vi "MCLB_FocusIndexArray_Tests.vi"(11 "error in":errorcluster) -> (15 "error out":errorcluster)   [LabVIEW 2016, in "DronaTest.lvlib"]
uses:
  DronaTest.lvlib
  APIs/Stimulus/ControlValue/SetValueAuto.vi
  APIs/Stimulus/ControlValue/Controls/MC Listbox/SetValueByArrayIndex.vi
  APIs/Assert/AssertControlValue/Controls/MC Listbox/AssertValueByArrayIndex.vi
  <vilib>/addons/_JKI Toolkits/Caraya/classes/Assert/Assert Error.vi
  <vilib>/addons/_JKI Toolkits/Caraya/classes/Assert/Assert Equal Value_Variant.vi
  <vilib>/addons/_JKI Toolkits/Caraya/classes/Test/Test.lvclass
  Drona.lvlib
  <vilib>/SLL Toolkit/SLL Debug/SLL Debug.lvlib
  <vilib>/addons/_JKI Toolkits/Caraya/classes/Assert/Assert.lvclass
  APIs/Stimulus/ControlValue/Controls/MC Listbox/StimulusMCListbox.lvlib
  APIs/Assert/AssertControlValue/Controls/MC Listbox/AssertMCListbox.lvlib
  APIs/Stimulus/ControlValue/ControlValue.lvlib
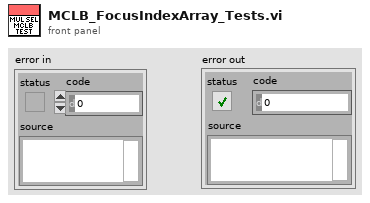
[diagram p1: front panel]
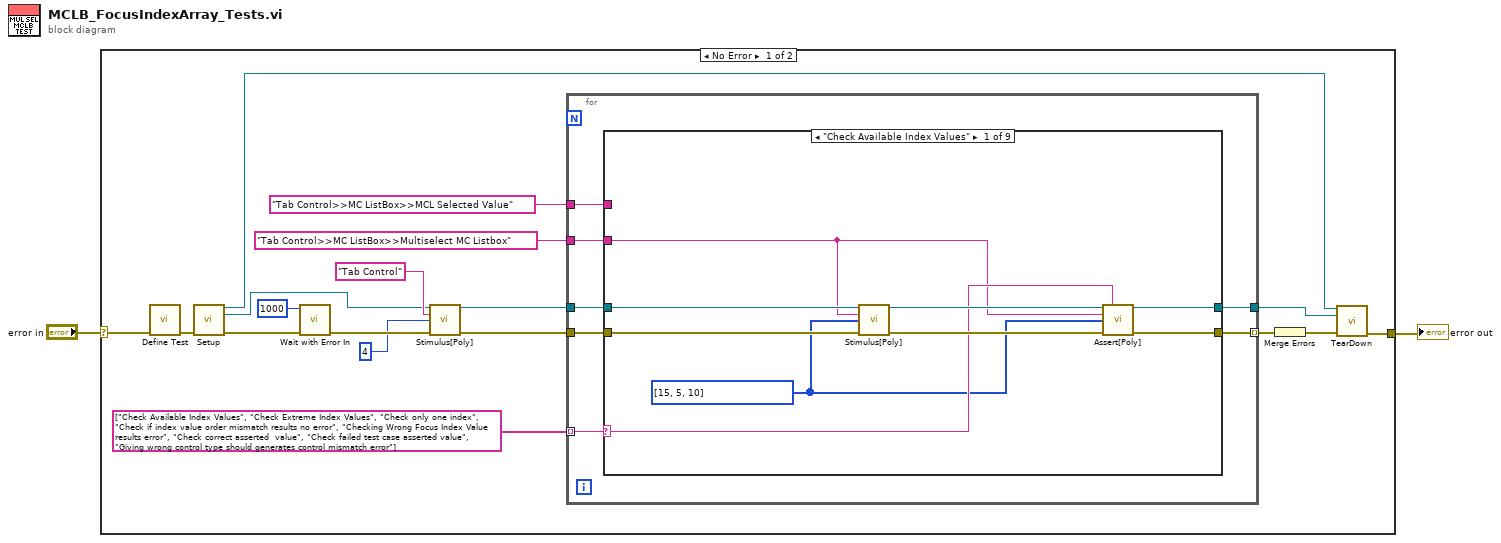
[diagram p0: block diagram]
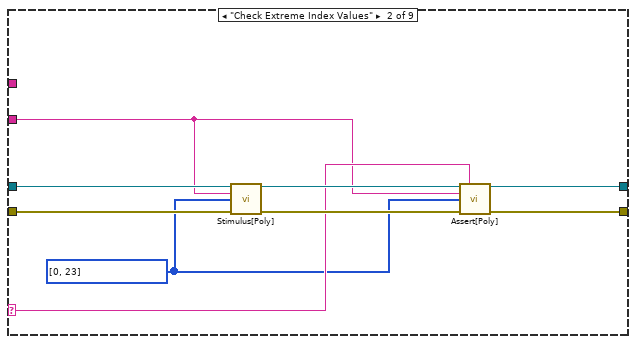
[diagram p2: hidden frame]
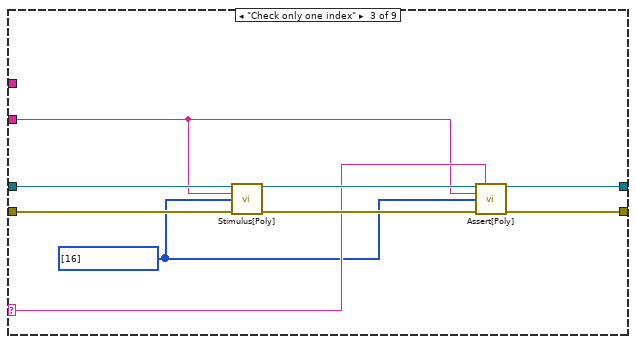
[diagram p3: hidden frame]
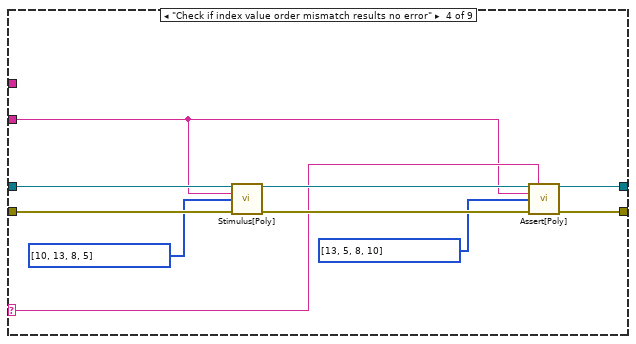
[diagram p4: hidden frame]
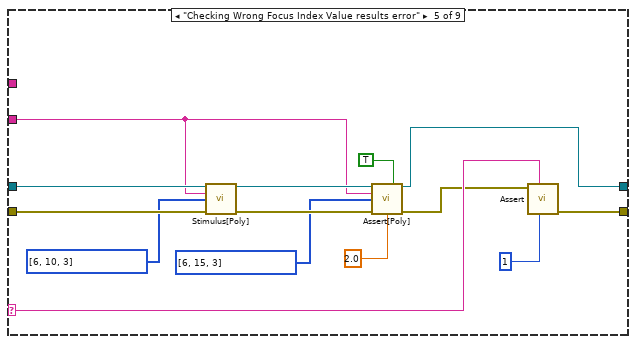
[diagram p5: hidden frame]
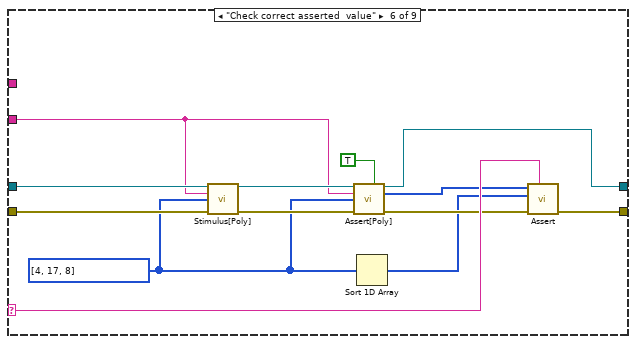
[diagram p6: hidden frame]
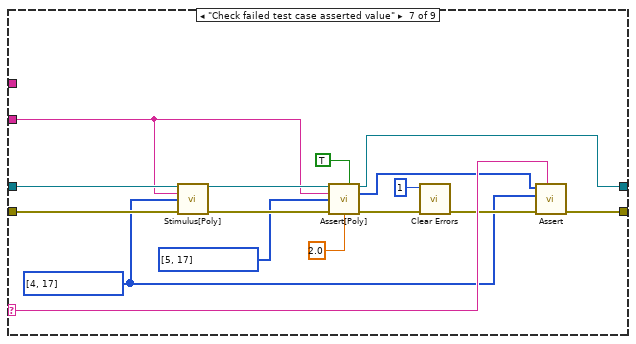
[diagram p7: hidden frame]
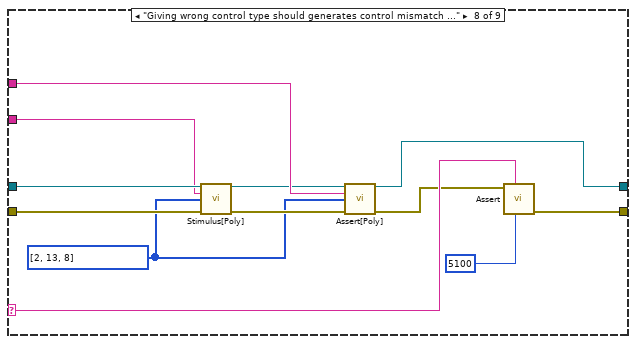
[diagram p8: hidden frame]
diagram:
  n1 = case shown="No Error" "error in" {
    selector: "error in" -> [w20 w122]
    tunnel: [w3 w122] -> w1
    frame No Error {
      n2 = call <vilib>:"Define Test.vi"("error in (no error)"=w20) -> ("error out"=w9:errorcluster)  [unwired: 9 in, 1 out]
      n3 = call "Setup.vi"("error in"=w9) -> ("Application Ref"=w5:refnum<vi>, "VI out"=w7:refnum<vi>, "error out"=w8:errorcluster)  [unwired: 12 in]
      n4 = call <vilib>:"Wait with Error In.vi"("error in (no error)"=w8, "milliseconds to wait"=u32 1000) -> ("error out"=w18:errorcluster)  [unwired: 9 in]
      n5 = call-poly "Stimulus[Poly].vi"("VI Reference In"=w7, "Control Path"="Tab Control", "Value (Signaling)"=4, "error in"=w18) -> ("VI Reference Out"=w14:refnum<vi>, "error out"=w17:errorcluster)  [unwired: 10 in]
      n6 = for {
        tunnel: w14 -> [w26]
        tunnel: "Tab Control>>MC ListBox>>Multiselect MC Listbox" ("Control Path") -> [w25]
        tunnel: "Tab Control>>MC ListBox>>MCL Selected Value" ("Control Path") -> [w24]
        tunnel: string[] ["Check Available Index Values", "Check Extreme Index Values", "Check only one index", "Check if index value order mismatch results no error", "Checking Wrong Focus Index Value results error", "Check correct asserted  value", "Check failed test case asserted value", "Giving wrong control type should generates control mismatch error"] -> [w22] mode=indexing
        tunnel: [w21] -> w4
        tunnel: w17 -> [w27]
        tunnel: [w23] -> w10 mode=indexing
        n7 = case shown="\"Check Available Index Values\"" w22 {
          selector: w22 -> [w30 w39 w48 w58 w77 w90 w106 w118 _]
          tunnel: w27 -> [w36 w45 w54 w64 w75 w89 w105 w113 w121]
          tunnel: w26 -> [w35 w44 w53 w63 w74 w88 w104 w111 w120]
          tunnel: w25 -> [w29 w38 w47 w57 w71 w85 w101 w109 _]
          tunnel: w24 -> [_ _ _ _ _ _ _ w115 _]
          tunnel: [w32 w41 w50 w60 w78 w91 w107 w119 w121] -> w23
          tunnel: [w31 w40 w49 w59 w70 w84 w100 w114 w120] -> w21
          frame "Check Available Index Values" {
            w28 = i32[] [15, 5, 10] ("Index Array")
            n8 = call-poly "Stimulus[Poly].vi"("VI Reference In"=w35, "Control Path"=w29, "Index Array"=w28, "Error In"=w36) -> ("VI Reference Out"=w33:refnum<vi>, "Error Out"=w34:errorcluster)  [unwired: 10 in]
            n9 = call-poly "Assert[Poly].vi"("VI Reference In"=w33, "Test Label"=w30, "Control Path"=w29, "Focus Item Index"=w28, "Error In"=w34) -> ("VI Reference Out"=w31:refnum<vi>, "Error Out"=w32:errorcluster)  [unwired: 8 in, 1 out]
          }
          frame "Check Extreme Index Values" {
            w37 = i32[] [0, 23] ("Index Array")
            n10 = call-poly "Stimulus[Poly].vi"("VI Reference In"=w44, "Control Path"=w38, "Index Array"=w37, "Error In"=w45) -> ("VI Reference Out"=w42:refnum<vi>, "Error Out"=w43:errorcluster)  [unwired: 10 in]
            n11 = call-poly "Assert[Poly].vi"("VI Reference In"=w42, "Test Label"=w39, "Control Path"=w38, "Focus Item Index"=w37, "Error In"=w43) -> ("VI Reference Out"=w40:refnum<vi>, "Error Out"=w41:errorcluster)  [unwired: 8 in, 1 out]
          }
          frame "Check only one index" {
            w46 = i32[] [16] ("Index Array")
            n12 = call-poly "Stimulus[Poly].vi"("VI Reference In"=w53, "Control Path"=w47, "Index Array"=w46, "Error In"=w54) -> ("VI Reference Out"=w51:refnum<vi>, "Error Out"=w52:errorcluster)  [unwired: 10 in]
            n13 = call-poly "Assert[Poly].vi"("VI Reference In"=w51, "Test Label"=w48, "Control Path"=w47, "Focus Item Index"=w46, "Error In"=w52) -> ("VI Reference Out"=w49:refnum<vi>, "Error Out"=w50:errorcluster)  [unwired: 8 in, 1 out]
          }
          frame "Check if index value order mismatch results no error" {
            n14 = call-poly "Stimulus[Poly].vi"("VI Reference In"=w63, "Control Path"=w57, "Index Array"=i32[] [10, 13, 8, 5], "Error In"=w64) -> ("VI Reference Out"=w61:refnum<vi>, "Error Out"=w62:errorcluster)  [unwired: 10 in]
            n15 = call-poly "Assert[Poly].vi"("VI Reference In"=w61, "Test Label"=w58, "Control Path"=w57, "Focus Item Index"=i32[] [13, 5, 8, 10] ("Index Array"), "Error In"=w62) -> ("VI Reference Out"=w59:refnum<vi>, "Error Out"=w60:errorcluster)  [unwired: 8 in, 1 out]
          }
          frame "Checking Wrong Focus Index Value results error" {
            n16 = call-poly "Stimulus[Poly].vi"("VI Reference In"=w74, "Control Path"=w71, "Index Array"=i32[] [6, 10, 3], "Error In"=w75) -> ("VI Reference Out"=w72:refnum<vi>, "Error Out"=w73:errorcluster)  [unwired: 10 in]
            n17 = call-poly "Assert[Poly].vi"("VI Reference In"=w72, "Assert Only? (F)"=TRUE, "Control Path"=w71, "Focus Item Index"=i32[] [6, 15, 3] ("Index Array"), "Error In"=w73, "Timeout(5 sec)"=2.0) -> ("VI Reference Out"=w70:refnum<vi>, "Error Out"=w69:errorcluster)  [unwired: 7 in, 1 out]
            n18 = call-poly <vilib>:"Assert.vi"("error code (1)"=1, "Label"=w77, "Error?"=w69) -> ("error out"=w78:errorcluster)  [unwired: 7 in, 1 out]
          }
          frame "Check correct asserted  value" {
            w80 = i32[] [4, 17, 8] ("Index Array")
            n19 = call-poly "Stimulus[Poly].vi"("VI Reference In"=w88, "Control Path"=w85, "Index Array"=w80, "Error In"=w89) -> ("VI Reference Out"=w86:refnum<vi>, "Error Out"=w87:errorcluster)  [unwired: 10 in]
            n20 = call-poly "Assert[Poly].vi"("VI Reference In"=w86, "Assert Only? (F)"=TRUE, "Control Path"=w85, "Focus Item Index"=w80, "Error In"=w87) -> ("VI Reference Out"=w84:refnum<vi>, "Asserted Value"=w82:i32[], "Error Out"=w83:errorcluster)  [unwired: 8 in]
            n21 = Sort 1D Array(array=w80) -> (sorted array=w79:i32[])
            n22 = call-poly <vilib>:"Assert.vi"("Label"=w90, "error in (no error)"=w83, "Y"=w79, "X"=w82) -> ("error out"=w91:errorcluster)  [unwired: 6 in, 1 out]
          }
          frame "Check failed test case asserted value" {
            w93 = i32[] [4, 17] ("Index Array")
            n23 = call-poly "Stimulus[Poly].vi"("VI Reference In"=w104, "Control Path"=w101, "Index Array"=w93, "Error In"=w105) -> ("VI Reference Out"=w102:refnum<vi>, "Error Out"=w103:errorcluster)  [unwired: 10 in]
            n24 = call-poly "Assert[Poly].vi"("VI Reference In"=w102, "Assert Only? (F)"=TRUE, "Control Path"=w101, "Focus Item Index"=i32[] [5, 17] ("Index Array"), "Error In"=w103, "Timeout(5 sec)"=2.0) -> ("VI Reference Out"=w100:refnum<vi>, "Asserted Value"=w94:i32[], "Error Out"=w99:errorcluster)  [unwired: 7 in]
            n25 = call <vilib>:"Clear Errors.vi"("error in (no error)"=w99, "specific error code to clear (0: all)"=1) -> ("error out"=w96:errorcluster)  [unwired: 4 in, 1 out]
            n26 = call-poly <vilib>:"Assert.vi"("Label"=w106, "error in (no error)"=w96, "Y"=w93, "X"=w94) -> ("error out"=w107:errorcluster)  [unwired: 6 in, 1 out]
          }
          frame "Giving wrong control type should generates control mismatch error" {
            w108 = i32[] [2, 13, 8] ("Index Array")
            n27 = call-poly "Stimulus[Poly].vi"("VI Reference In"=w111, "Control Path"=w109, "Index Array"=w108, "Error In"=w113) -> ("VI Reference Out"=w110:refnum<vi>, "Error Out"=w112:errorcluster)  [unwired: 10 in]
            n28 = call-poly "Assert[Poly].vi"("VI Reference In"=w110, "Control Path"=w115, "Focus Item Index"=w108, "Error In"=w112) -> ("VI Reference Out"=w114:refnum<vi>, "Error Out"=w116:errorcluster)  [unwired: 9 in, 1 out]
            n29 = call-poly <vilib>:"Assert.vi"("error code (1)"=5100, "Label"=w118, "Error?"=w116) -> ("error out"=w119:errorcluster)  [unwired: 7 in, 1 out]
          }
          frame Default {
          }
        }
      }
      n30 = Merge Errors(w10) -> (w6:errorcluster)
      n31 = call "TearDown.vi"("Application Ref"=w5, "VI in"=w4, "error in (no error)"=w6) -> ("error out"=w3:errorcluster)  [unwired: 12 in]
    }
    frame Error {
    }
  }
  "error out" <- w1
